vi "query NR Operation Band.vi"(8 "error in (no error)":errorcluster, 10 "Selected CC Argements":T1, 11 "Anritsu Call Box in":refnum<class "Anritsu Call Box.lvclass">) -> (0 "error out":errorcluster, 2 "Operation Band":u32, 3 "Anritsu Call Box out":refnum<class "Anritsu Call Box.lvclass">)   [LabVIEW 2023, in "ANRITSU Call Box.lvlib" / "Anritsu Call Box.lvclass"]
uses:
  Anritsu Call Box.lvclass
  Type Definition/NR Selected CC Type Arguments.ctl
  ANRITSU Call Box.lvlib
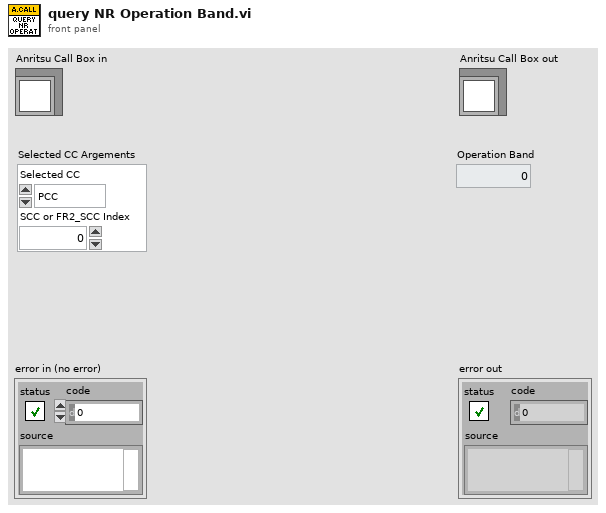
[diagram p1: front panel]
types:
  T1 = typedef "ANRITSU Call Box.lvlib/NR Selected CC Type Arguments.ctl" = cluster{"Selected CC":enum16{"PCC", "SCC", "FR2_PCC", "FR2_SCC"}, "SCC or FR2_SCC Index":u32}
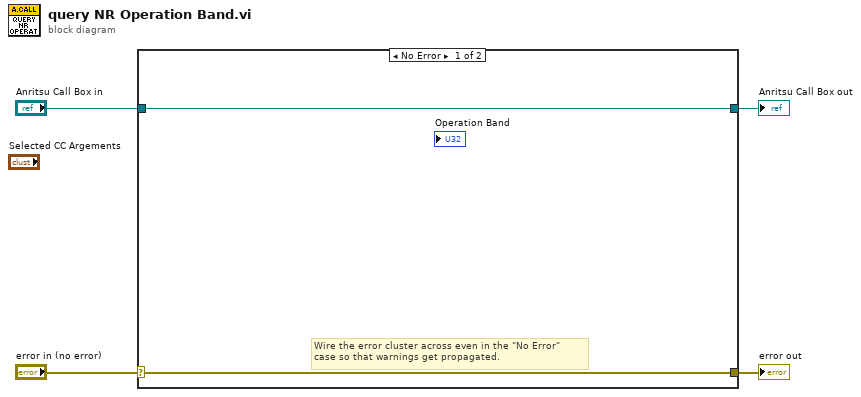
[diagram p0: block diagram]
diagram:
  n1 = case shown="No Error" "error in (no error)" {
    selector: "error in (no error)" -> [w5 w8]
    tunnel: [w5 w8] -> w3
    tunnel: [w6 w7] -> w1
    tunnel: "Anritsu Call Box in" -> [w6 w7]
    frame No Error {
      # "Wire the error cluster across even in the \"No Error\"\ncase so that warnings get propagated."
    }
    frame Error {
    }
  }
  "error out" <- w3
  "Anritsu Call Box out" <- w1
